vi "Measurement Logic.vi"(8 "error in":errorcluster, 9 "measurement configuration":T2 {"Baudrate" format="%x"; "FD Baudrate" format="%x"}, 10 "measure call context in":refnum<class "Measure Call Context.lvclass">) -> (0 "error out":errorcluster, 1 "measurement results":T1, 2 "measure call context out":refnum<class "Measure Call Context.lvclass">)   [LabVIEW 2025, in "CAN-LIN Raw Bus Capture.lvclass"]
doc: "Contains the core logic for executing the measurement."
uses:
  CAN-LIN Raw Bus Capture.lvclass
  <vilib>/Plug-In SDKs/Measurements/Measure Call Context/Measure Call Context.lvclass
  Measurement Configuration.ctl
  CAN-LIN Raw Bus Capture UI/Toggle.ctl
  Measurement Results.ctl
  CAN-LIN Raw Bus Capture.lvclass/CAN-LIN Raw Bus Capture.ctl
  <vilib>/xnet/xnet.llb/XNET Read (Frame CAN).vi
  <vilib>/xnet/xnet.llb/XNET Read (State CAN Comm).vi
  <vilib>/xnet/xnet.llb/XNET Read (State LIN Comm).vi
  <vilib>/xnet/xnet.llb/XNET Read (Frame LIN).vi
  session-management/xnetCAN/Session Management xnetCAN.lvlib
  <vilib>/Plug-In SDKs/Clients/Session Management V1/Session Reservation/Session Reservation.lvclass
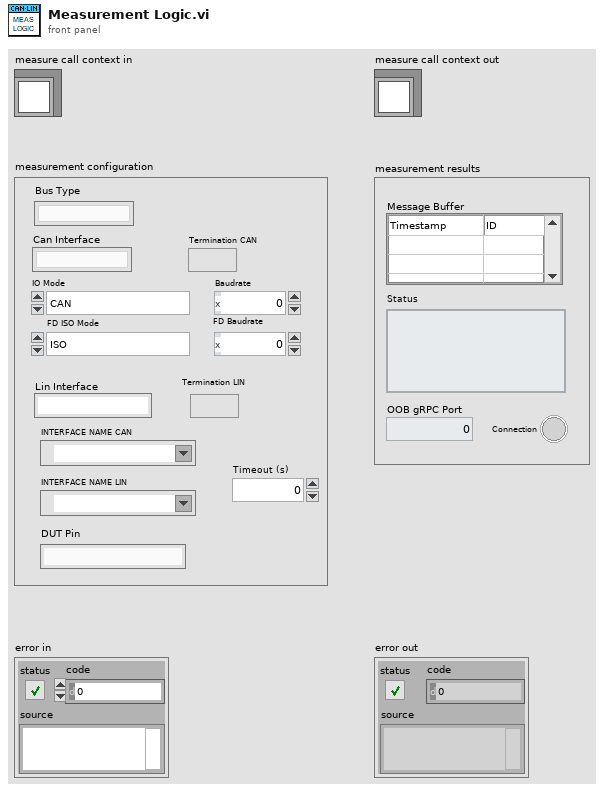
[diagram p1: front panel]
types:
  T1 = typedef "CAN-LIN Raw Bus Capture.lvclass/Measurement Results.ctl" = cluster{"Message Buffer":string[][], "Status":string, "OOB gRPC Port":i32, "Connection":bool}
  T2 = typedef "CAN-LIN Raw Bus Capture.lvclass/Measurement Configuration.ctl" = cluster{"Termination CAN":T3, "FD Baudrate":u32, "Baudrate":u32, "FD ISO Mode":enum32{"ISO", "Legacy ISO", "Non-ISO"}, "IO Mode":enum32{"CAN", "CAN FD", "CAN FD + BRS"}, "Termination LIN":T3, "Can Interface":string, "Lin Interface":string, "Bus Type":string, "INTERFACE NAME CAN":refnum<k21>, "INTERFACE NAME LIN":refnum<k21>, "Timeout (s)":u32, "DUT Pin":string}
  T3 = typedef "Toggle.ctl" = bool
  T4 = typedef "Session Management xnetCAN.lvlib/Connection with Session.ctl" = cluster{"connection":T5, "session":string}
  T5 = typedef "NI Session Management V1 Client.lvlib/Session Reservation.lvclass/Connection.ctl" = cluster{"pin or relay name":string, "site":i32, "instrument type id":string, "channel":string}
  T6 = typedef "XNET Frame CAN.ctl" = cluster{"timestamp":timestamp, "payload":u8[], "identifier":u32, "type":T7, "extended?":bool, "echo?":bool}
  T7 = typedef "XNET Frame Type CAN.ctl" = u8
  T8 = typedef "XNET CAN Comm.ctl" = cluster{"fault code":i32, "fault?":bool, "communication state":T9, "last error":T10, "receive error counter":u8, "transmit error counter":u8, "transceiver error?":bool, "sleep?":bool}
  T9 = typedef "XNET CAN Comm State.ctl" = u8
  T10 = typedef "XNET CAN Last Err.ctl" = u8
  T11 = typedef "XNET Frame LIN.ctl" = cluster{"timestamp":timestamp, "payload":u8[], "identifier":u32, "type":T12, "event ID":u8, "event slot?":bool, "echo?":bool}
  T12 = typedef "XNET Frame Type LIN.ctl" = u8
  T13 = typedef "XNET LIN Comm.ctl" = cluster{"fault code":i32, "fault?":bool, "communication state":T14, "last error":T15, "last error received":u8, "last error expected":u8, "last error identifier":u8, "sleep?":bool, "transceiver ready?":bool, "schedule index":u8}
  T14 = typedef "XNET LIN Comm State.ctl" = u8
  T15 = typedef "XNET LIN Last Err.ctl" = u8
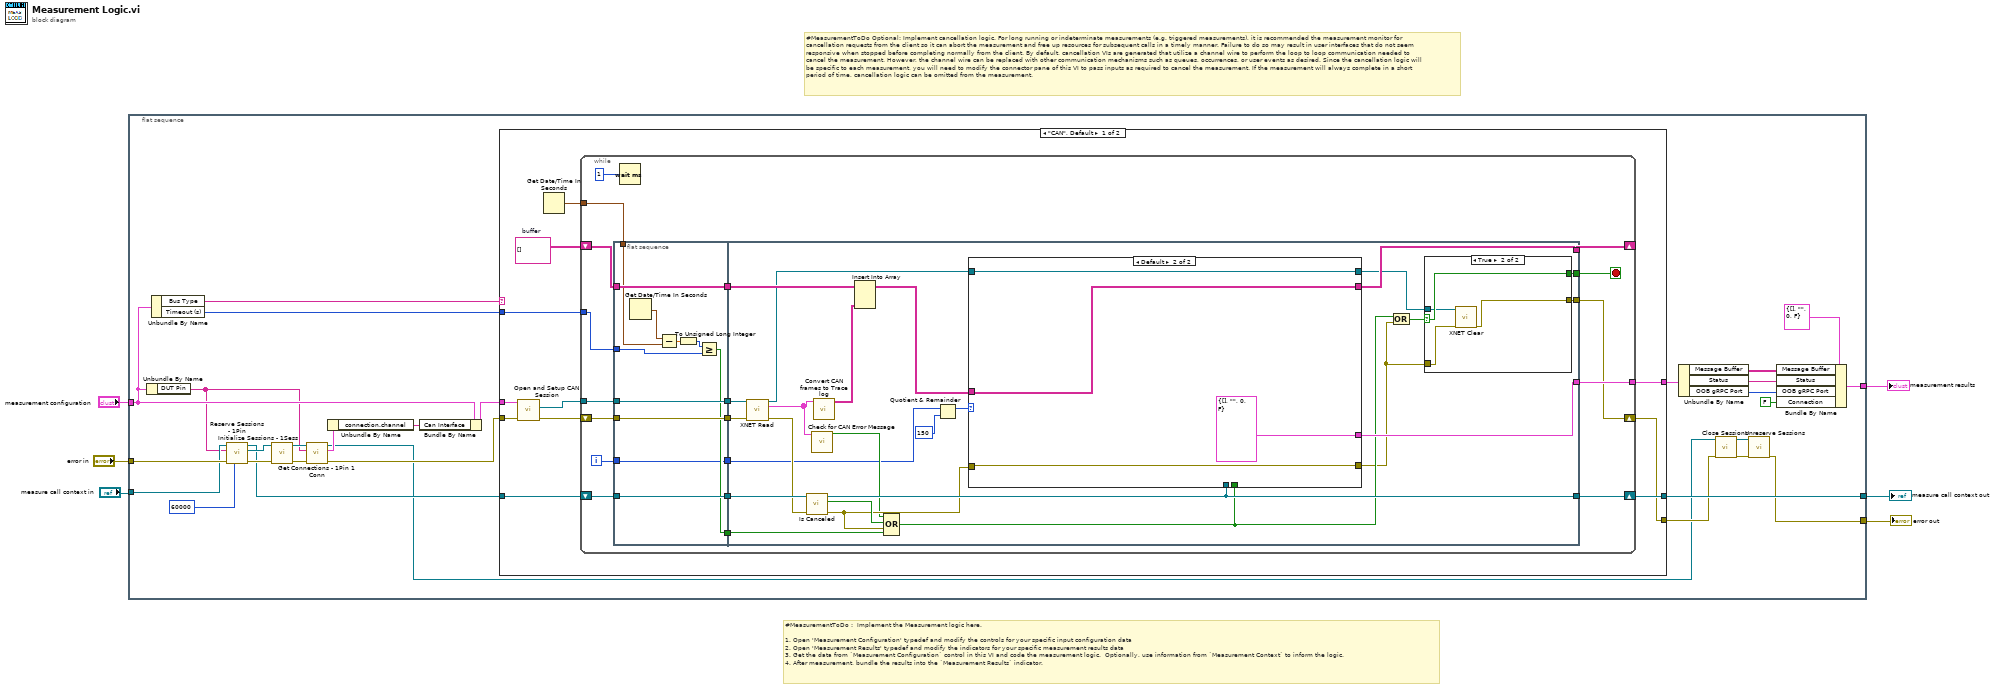
[diagram p0: block diagram]
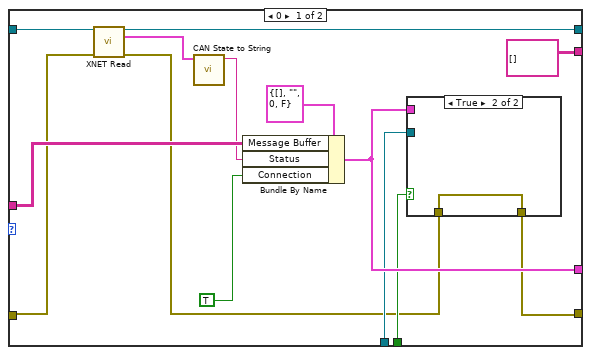
[diagram p2: hidden frame]
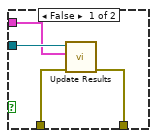
[diagram p3: hidden frame]
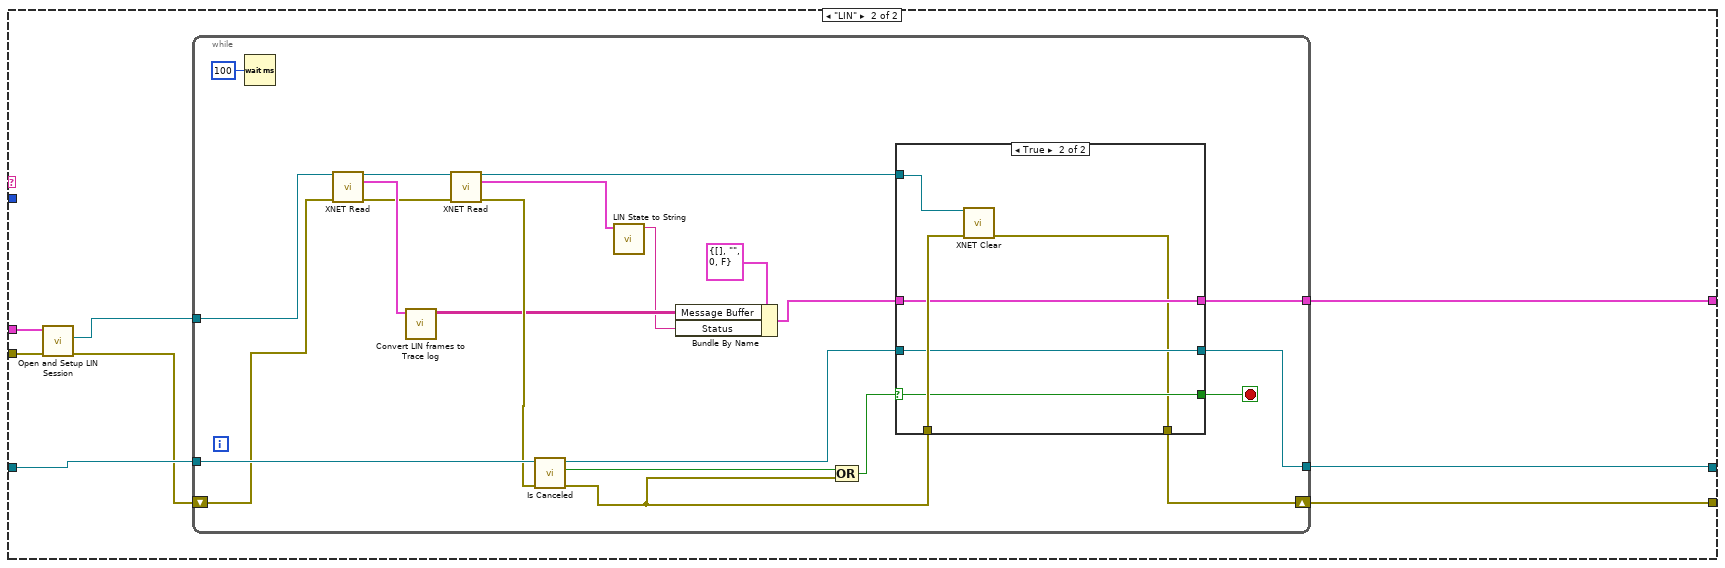
[diagram p5: hidden frame]
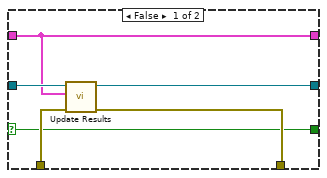
[diagram p6: hidden frame]
diagram:
  # "#MeasurementToDo Optional: Implement cancellation logic. For long running or indeterminate measurements (e.g. triggered measurements), it is recommended the measurement monitor for cancellation requests from the client so it can abort the measurement and free up resources for subsequent calls in a timely manner. Failure to do so may result in user interfaces that do not seem responsive when stopped before completing normally from the client. By default, cancellation VIs are generated that utilize a channel wire to perform the loop to loop communication needed to cancel the measurement. However, the channel wire can be replaced with other communication mechanisms such as queues, occurrences, or user events as desired. Since the cancellation logic will be specific to each measurement, you will need to modify the connector pane of this VI to pass inputs as required to cancel the measurement. If the measurement will always complete in a short period of time, cancellation logic can be omitted from the measurement."
  # "#MeasurementToDo :  Implement the Measurement logic here.\n\n1. Open 'Measurement Configuration' typedef and modify the controls for your specific input configuration data\n2. Open 'Measurement Results' typedef and modify the indicators for your specific measurement results data\n3. Get the data from `Measurement Configuration` control in this VI and code the measurement logic.  Optionally, use information from `Measurement Context` to inform the logic.\n4. After measurement, bundle the results into the `Measurement Results` indicator."
  n1 = flat-sequence {
    tunnel: "measurement configuration" -> [w16]
    tunnel: [w32] -> w5
    tunnel: "error in" -> [w20]
    tunnel: "measure call context in" -> [w18]
    tunnel: [w8] -> w3
    tunnel: [w34] -> w2
    frame #0 {
      n2 = Unbundle By Name(w16) -> ("DUT Pin"=w15:string)
      n3 = Unbundle By Name(w16) -> ("Bus Type"=w35:string, "Timeout (s)"=w26:u32)
      n4 = call <vilib>:"Reserve Sessions - 1Pin.vi"("timeout (ms)"=60000 ("timeout in milliseconds"), "error in"=w20, "pin or relay name"=w15, "measurement context in"=w18) -> ("error out"=w23:errorcluster, "session reservation out"=w22:refnum<class "Session Reservation.lvclass">, "measurement context out"=w17:refnum<class "Measure Call Context.lvclass">)  [unwired: 5 in]
      n5 = call "Initialize Sessions - 1Sess.vi"("error in"=w23, "session reservation in"=w22) -> ("error out"=w25:errorcluster, "session reservation out"=w24:refnum<class "Session Reservation.lvclass">)  [unwired: 6 in, 2 out]
      n6 = call "Get Connections - 1Pin 1 Conn.vi"("error in"=w25, "pin or relay name"=w15, "session reservation in"=w24) -> ("error out"=w19:errorcluster, "connection"=w14:T4, "session reservation out"=w7:refnum<class "Session Reservation.lvclass">)  [unwired: 6 in]
      n7 = Unbundle By Name(w14) -> ("connection.channel"=w12:string)
      n8 = Bundle By Name(cluster=w16, "Can Interface"=w12) -> (w13:T2)
      n9 = case shown="\"CAN\", Default" w35 {
        tunnel: w13 -> [w44 w132]
        tunnel: w17 -> [w43 w135]
        tunnel: w19 -> [w42 w134]
        tunnel: [w41 w136] -> w33
        tunnel: [w40 w138] -> w34
        tunnel: [w39 w137] -> w9
        tunnel: w26 -> [w36 _]
        frame "CAN", Default {
          w38 = string[][] []  # buffer
          n10 = call "Open and Setup CAN Session.vi"("error in"=w42, "measurement configuration"=w44) -> ("error out"=w45:errorcluster, "session out"=w46:refnum<k21>)  [unwired: 8 in]
          n11 = Get Date/Time In Seconds() -> (seconds since 1Jan1904=w37:timestamp)
          n12 = while {
            tunnel: [w60] -> w41
            shift-right: [w56] -> w39
            shift-left: w45 -> [w63]
            tunnel: w46 -> [w62]
            shift-right: [w58] -> w40
            shift-left: w43 -> [w64]
            shift-right: [w57] -> _
            shift-left: w38 -> [w59]
            tunnel: w37 -> [w51]
            tunnel: w36 -> [w50]
            i -> [w47]
            stop <- w61 stop-if-true
            n13 = flat-sequence {
              tunnel: w59 -> [w73]
              tunnel: w62 -> [w74]
              tunnel: w63 -> [w75]
              tunnel: w64 -> [w76]
              tunnel: [w76] -> w55
              tunnel: [w75] -> w54
              tunnel: [w74] -> w53
              tunnel: [w73] -> w52
              tunnel: w51 -> [w71]
              tunnel: w50 -> [w69]
              tunnel: [w68] -> w49
              tunnel: [w66] -> w48
              tunnel: w47 -> [w66]
              tunnel: [w98] -> w61
              tunnel: [w95] -> w60
              tunnel: [w90] -> w58
              tunnel: [w87] -> w57
              tunnel: [w86] -> w56
              tunnel: w55 -> [w101]
              tunnel: w54 -> [w100]
              tunnel: w53 -> [w99]
              tunnel: w52 -> [w92]
              tunnel: w49 -> [w78]
              tunnel: w48 -> [w77]
              frame #0 {
                n14 = Get Date/Time In Seconds() -> (seconds since 1Jan1904=w72:timestamp)
                n15 = Subtract(x=w72, y=w71) -> (x-y=w70:dbl)
                n16 = To Unsigned Long Integer(number=w70) -> (unsigned 32bit integer=w67:u32)
                n17 = Greater Or Equal?(x=w67, y=w69) -> (x >= y?=w68:bool)
              }
              frame #1 {
                n18 = call-poly <vilib>:"XNET Read.vi"("session in"=w99, "error in (no error)"=w100) -> ("session out"=w88:refnum<k21>, "data"=w79:T6[], "error out"=w96:errorcluster)  [unwired: 10 in, 1 out]
                n19 = call <vilib>:"Is Canceled.vi"("error in"=w96, "measure call context in"=w101) -> ("error out"=w89:errorcluster, "is canceled?"=w97:bool, "measure call context out"=w90:refnum<class "Measure Call Context.lvclass">)  [unwired: 7 in]
                n20 = call "Check for CAN Error Message.vi"("data"=w79) -> ("Error"=w81:bool)  [unwired: 9 in, 1 out]
                n21 = call "Convert CAN frames to Trace log.vi"("can frames in"=w79) -> ("trace out"=w80:string[][])  [unwired: 10 in]
                n22 = Insert Into Array(array=w92, new element=w80) -> (w91:string[][])  [unwired: 2 in]
                n23 = Compound Arithmetic op=OR(w81, w97, w89, w78) -> (w84:bool)
                n24 = Quotient & Remainder(x=w77, y=150) -> (x-y*floor(x/y)=w93:i32)  [unwired: 1 out]
                n25 = case shown="Default" w93 {
                  tunnel: [w114 T1 {"Message Buffer"=[], "Status"="", "OOB gRPC Port"=0, "Connection"=FALSE} ("Measurement Results")] -> w95
                  tunnel: w91 -> [w109 w123]
                  tunnel: w84 -> [w113 _]
                  tunnel: w90 -> [w112 _]
                  tunnel: w89 -> [w107 w124]
                  tunnel: w88 -> [w108 w121]
                  tunnel: [w111 w124] -> w83
                  tunnel: [string[][] [] ("buffer") w123] -> w87
                  tunnel: [w102 w121] -> w85
                  frame 0 {
                    n26 = call-poly <vilib>:"XNET Read.vi"("session in"=w108, "error in (no error)"=w107) -> ("session out"=w102:refnum<k21>, "CAN comm"=w105:T8, "error out"=w106:errorcluster)  [unwired: 11 in]
                    n27 = call "CAN State to String.vi"("CAN comm in"=w105) -> ("string out"=w104:string)  [unwired: 10 in]
                    n28 = Bundle By Name(cluster=T1 {"Message Buffer"=[], "Status"="", "OOB gRPC Port"=0, "Connection"=FALSE} ("Measurement Results"), "Message Buffer"=w109, "Status"=w104, "Connection"=TRUE) -> (w114:T1)
                    n29 = case shown="True" w113 {
                      tunnel: w112 -> [w119 _]
                      tunnel: w106 -> [w118 w120]
                      tunnel: [w117 w120] -> w111
                      tunnel: w114 -> [w116 _]
                      frame False {
                        n30 = call <vilib>:"Update Results.vi"("error in"=w118, "measurement results"=w116, "measure call context in"=w119) -> ("error out"=w117:errorcluster)  [unwired: 7 in, 1 out]
                      }
                      frame True {
                      }
                    }
                  }
                  frame Default {
                  }
                }
                n31 = Compound Arithmetic op=OR(w84, w83) -> (w82:bool)
                n32 = case shown="True" w82 {
                  selector: w82 -> [w126 w130]
                  tunnel: [w126 w130] -> w98
                  tunnel: w83 -> [w125 w128]
                  tunnel: [w125 w127] -> w86
                  tunnel: w85 -> [_ w129]
                  frame False {
                  }
                  frame True {
                    n33 = call <vilib>:"XNET Clear.vi"("session in"=w129, "error in (no error)"=w128) -> ("error out"=w127:errorcluster)  [unwired: 13 in]
                  }
                }
              }
            }
            n34 = Wait (ms)(milliseconds to wait=u32 1) -> ()  [unwired: 1 out]
          }
        }
        frame "LIN" {
          n35 = call "Open and Setup LIN Session.vi"("error in"=w134, "measurement configuration"=w132) -> ("error out"=w133:errorcluster, "session out"=w131:refnum<k21>)  [unwired: 8 in]
          n36 = while {
            tunnel: [w146] -> w136
            tunnel: w135 -> [w159]
            tunnel: [w156] -> w138
            shift-right: [w152] -> w137
            shift-left: w133 -> [w158]
            tunnel: w131 -> [w153]
            stop <- w147 stop-if-true
            n37 = Wait (ms)(milliseconds to wait=u32 100) -> ()  [unwired: 1 out]
            n38 = call-poly <vilib>:"XNET Read.vi"("session in"=w153, "error in (no error)"=w158) -> ("session out"=w142:refnum<k21>, "data"=w144:T11[], "error out"=w139:errorcluster)  [unwired: 10 in, 1 out]
            n39 = call "Convert LIN frames to Trace log.vi"("lin frames in"=w144) -> ("trace out"=w143:string[][])  [unwired: 10 in]
            n40 = call-poly <vilib>:"XNET Read.vi"("session in"=w142, "error in (no error)"=w139) -> ("session out"=w155:refnum<k21>, "LIN comm"=w141:T13, "error out"=w148:errorcluster)  [unwired: 11 in]
            n41 = call <vilib>:"Is Canceled.vi"("error in"=w148, "measure call context in"=w159) -> ("error out"=w151:errorcluster, "is canceled?"=w150:bool, "measure call context out"=w157:refnum<class "Measure Call Context.lvclass">)  [unwired: 7 in]
            n42 = call "LIN State to String.vi"("LIN comm in"=w141) -> ("string out"=w140:string)  [unwired: 10 in]
            n43 = Bundle By Name(cluster=T1 {"Message Buffer"=[], "Status"="", "OOB gRPC Port"=0, "Connection"=FALSE} ("Measurement Results"), "Message Buffer"=w143, "Status"=w140) -> (w154:T1)
            n44 = Compound Arithmetic op=OR(w150, w151) -> (w149:bool)
            n45 = case shown="True" w149 {
              selector: w149 -> [w162 w169]
              tunnel: w157 -> [w166 w170]
              tunnel: w151 -> [w165 w172]
              tunnel: [w164 w167] -> w152
              tunnel: [w163 w170] -> w156
              tunnel: w155 -> [_ w171]
              tunnel: w154 -> [w161 w168]
              tunnel: [w162 w169] -> w147
              tunnel: [w161 w168] -> w146
              frame False {
                n46 = call <vilib>:"Update Results.vi"("error in"=w165, "measurement results"=w161, "measure call context in"=w166) -> ("error out"=w164:errorcluster, "measure call context out"=w163:refnum<class "Measure Call Context.lvclass">)  [unwired: 7 in]
              }
              frame True {
                n47 = call <vilib>:"XNET Clear.vi"("session in"=w171, "error in (no error)"=w172) -> ("error out"=w167:errorcluster)  [unwired: 13 in]
              }
            }
          }
        }
      }
      n48 = Unbundle By Name(w33) -> ("Message Buffer"=w30:string[][], "Status"=w29:string, "OOB gRPC Port"=w27:i32)
      n49 = call <vilib>:"Close Sessions.vi"("error in"=w9, "session reservation in"=w7) -> ("error out"=w11:errorcluster, "session reservation out"=w10:refnum<class "Session Reservation.lvclass">)  [unwired: 8 in]
      n50 = call <vilib>:"Unreserve Sessions.vi"("error in"=w11, "session reservation in"=w10) -> ("error out"=w8:errorcluster)  [unwired: 9 in]
      n51 = Bundle By Name(cluster=T1 {"Message Buffer"=[], "Status"="", "OOB gRPC Port"=0, "Connection"=FALSE} ("Measurement Results"), "Message Buffer"=w30, "Status"=w29, "OOB gRPC Port"=w27, "Connection"=FALSE) -> (w32:T1)
    }
  }
  "error out" <- w3
  "measure call context out" <- w2
  "measurement results" <- w5
